vi "Live Image.vi"(8 "error in (no error)":errorcluster, 10 "Live.Data":T1, 11 "ImageHandler:Varex-ImageHandler in":refnum<class "Varex-ImageHandler.lvclass">) -> (0 "error out":errorcluster, 3 "ImageHandler:Varex-ImageHandler out":refnum<class "Varex-ImageHandler.lvclass">)   [LabVIEW 2022 SP3, in "ImageHandler.lvlib" / "Varex-ImageHandler.lvclass"]
uses:
  Varex-ImageHandler.lvclass
  Varex-ImageHandler.lvclass/Varex-ImageHandler.ctl
  VarexWrapperLvLib/VarexWrapper.lvlib
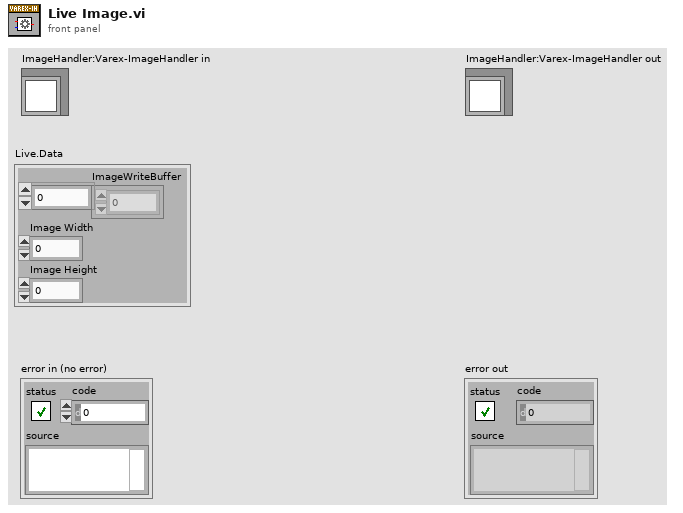
[diagram p1: front panel]
types:
  T1 = cluster{"ImageWriteBuffer":u16[], "Image Width":i32, "Image Height":i32}
  T2 = enum32{"Map Pixel Pointer", "Unmap Pixel Pointer", "Get Pixels Infos"}
  T3 = typedef "IMAQ Image.ctl" = refnum<image>
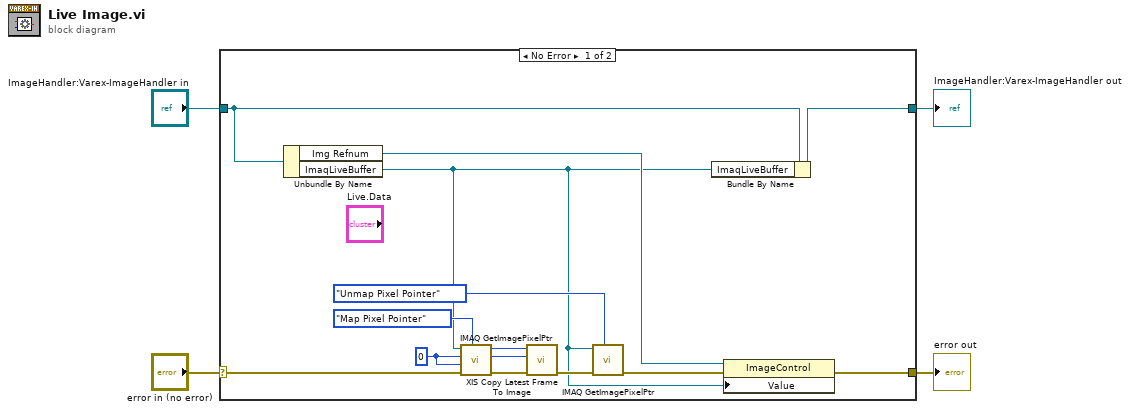
[diagram p0: block diagram]
diagram:
  n1 = case shown="No Error" "error in (no error)" {
    selector: "error in (no error)" -> [w17 w20]
    tunnel: [w16 w20] -> w3
    tunnel: [w6 w19] -> w1
    tunnel: "ImageHandler:Varex-ImageHandler in" -> [w18 w19]
    frame No Error {
      w11 = 0 ("X Coordinate")
      n2 = Unbundle By Name(w18) -> ("Img Refnum"=w15:refnum<vi>, "ImaqLiveBuffer"=w5:T3)
      n3 = call "IMAQ GetImagePixelPtr"("Function"=T2."Map Pixel Pointer", "error in (no error)"=w17, "Y Coordinate"=w11, "X Coordinate"=w11, "Image"=w5) -> ("error out"=w14:errorcluster, "LineWidth(Pixels)"=w7:i32, "Pixel Pointer out"=w8:u64)  [unwired: 1 in, 3 out]
      n4 = call "XIS Copy Latest Frame To Image.vi"("error in (no error)"=w14, "LVLineWidthPixels"=w7, "LVImagePtr"=w8) -> ("error out"=w12:errorcluster)  [unwired: 7 in, 1 out]
      n5 = call "IMAQ GetImagePixelPtr"("Function"=T2."Unmap Pixel Pointer", "error in (no error)"=w12, "Image"=w5) -> ("error out"=w13:errorcluster)  [unwired: 3 in, 5 out]
      n6 = Bundle By Name(cluster=w18, "ImaqLiveBuffer"=w5) -> (w6:refnum<class "Varex-ImageHandler.lvclass">)
      n7 = property class="ImageControl"(reference=w15, error in=w13, "Value"=w5) -> (error out=w16:errorcluster)  [unwired: 1 out]
    }
    frame Error {
    }
  }
  "error out" <- w3
  "ImageHandler:Varex-ImageHandler out" <- w1
